vi "VIH HelpGen - Build Object Description for HTML.vi"(7 "Ena \"No Description\" message (F)":bool, 8 "Generate \"HTML Description\" (T)":bool=TRUE, 9 "Custom Description":string, 10 "Default Description":string, 11 "DscrMode":T2) -> (0 "HTML Tagset allowed":T1(ring), 2 "Description HTML out":string)   [LabVIEW 2014]
doc: "::: VI Helpeks :::\nCopyright (c) 2000-2026 Konstantin Shifershteyn. All rights reserved."
uses:
  _VIH HelpGen.llb/VIH HelpGen Typedef - Enum - Description Mode.ctl
panel:
  in  "Use Descripion Terminator (T)":bool=TRUE
  # "VI Helpeks\nCopyright (c) 2012-2026 Konstantin Shifershteyn"
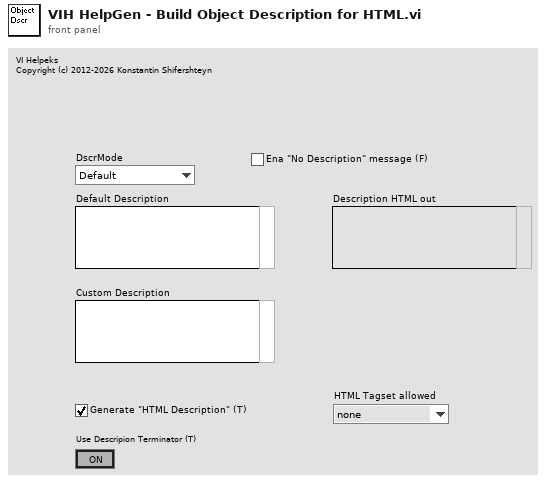
[diagram p1: front panel]
types:
  T1 = enum16{"none", "LV description", "VH minimum", "VH extended"}
  T2 = typedef "VIH HelpGen Typedef - Enum - Description Mode.ctl" = enum16{"Default", "Description", "Description1", "Description2", "Custom", "None"}
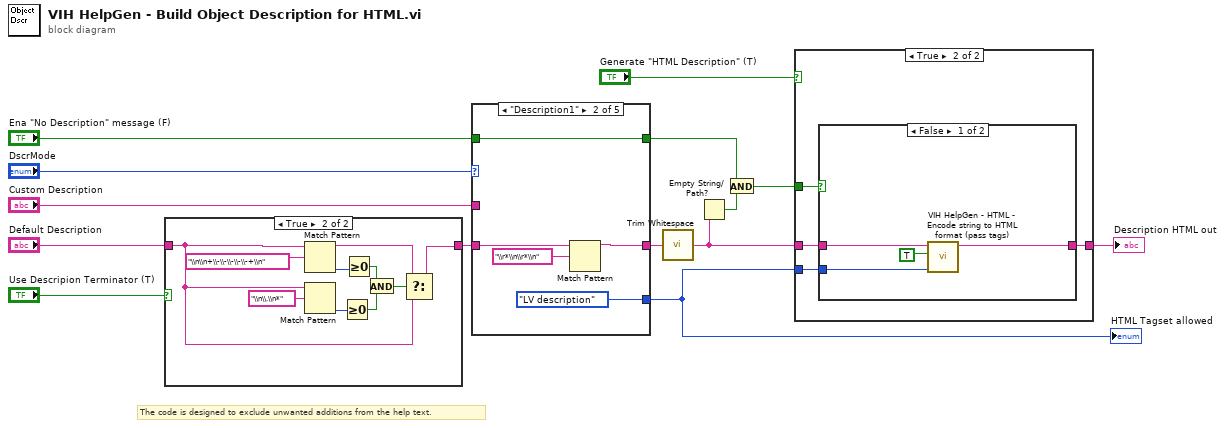
[diagram p0: block diagram]
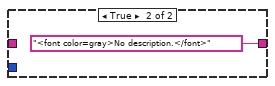
[diagram p4: hidden frame]
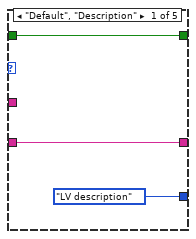
[diagram p5: hidden frame]
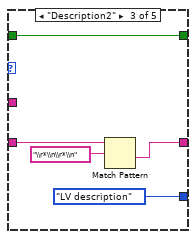
[diagram p6: hidden frame]
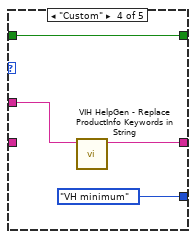
[diagram p7: hidden frame]
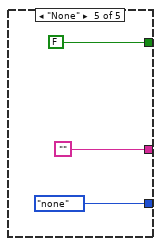
[diagram p8: hidden frame]
diagram:
  # "The code is designed to exclude unwanted additions from the help text."
  n1 = case shown="True" "Use Descripion Terminator (T)" {
    tunnel: "Default Description" -> [w15 w16]
    tunnel: [w15 w17] -> w2
    frame False {
    }
    frame True {
      n2 = Match Pattern(string=w16, regular expression="\\n\\n+\\-\\-\\-\\-\\-+\\n") -> (before substring=w19:string, offset past match=w23:i32)  [unwired: 1 in, 2 out]
      n3 = Match Pattern(string=w16, regular expression="\\n\\.\\n*") -> (offset past match=w22:i32)  [unwired: 1 in, 3 out]
      n4 = Greater Or Equal To 0?(x=w22) -> (x >= 0?=w20:bool)
      n5 = Greater Or Equal To 0?(x=w23) -> (x >= 0?=w21:bool)
      n6 = And(x=w21, y=w20) -> (x .and. y?=w18:bool)
      n7 = Select(t=w19, s=w18, f=w16) -> (s? t:f=w17:string)
    }
  }
  n8 = case shown="\"Description1\"" "DscrMode" {
    tunnel: w2 -> [w28 w33 w38 _ _]
    tunnel: [w28 w32 w35 w40 ""] -> w14
    tunnel: "Custom Description" -> [_ _ _ w39 _]
    tunnel: [w27 w31 w36 w42 FALSE] -> w7
    tunnel: "Ena \"No Description\" message (F)" -> [w27 w31 w36 w42 _]
    tunnel: [T1."LV description" ("Tag set") T1."LV description" ("Tag set") T1."LV description" ("Tag set") T1."VH minimum" ("Tag set") T1."none" ("Tag set")] -> w5
    frame "Default", "Description" {
    }
    frame "Description1" {
      n9 = Match Pattern(string=w33, regular expression="\\r*\\n\\r*\\n") -> (before substring=w32:string)  [unwired: 1 in, 3 out]
    }
    frame "Description2" {
      n10 = Match Pattern(string=w38, regular expression="\\r*\\n\\r*\\n") -> (after substring=w35:string)  [unwired: 1 in, 3 out]
    }
    frame "Custom" {
      n11 = call "VIH HelpGen - Replace ProductInfo Keywords in String.vi"("String in"=w39) -> ("String out"=w40:string)  [unwired: 10 in]
    }
    frame "None" {
    }
  }
  "HTML Tagset allowed" <- w5
  n12 = call <vilib>:"Trim Whitespace.vi"("string"=w14) -> ("trimmed string"=w8:string)  [unwired: 1 in]
  n13 = Empty String/Path?(string/path=w8) -> (empty?=w10:bool)
  n14 = And(x=w7, y=w10) -> (x .and. y?=w9:bool)
  n15 = case shown="True" "Generate \"HTML Description\" (T)" {
    tunnel: [w46 w50] -> w11
    tunnel: w9 -> [_ w49]
    tunnel: w8 -> [w46 w48]
    tunnel: w5 -> [_ w47]
    frame False {
    }
    frame True {
      n16 = case shown="False" w49 {
        tunnel: [w54 "<font color=gray>No description.</font>"] -> w50
        tunnel: w48 -> [w53 _]
        tunnel: w47 -> [w52 _]
        frame False {
          n17 = call "VIH HelpGen - HTML - Encode string to HTML format (pass tags).vi"("HTML Tagset allowed"=w52, "Reject CR (F)"=TRUE, "string"=w53) -> ("HTML string"=w54:string)  [unwired: 8 in]
        }
        frame True {
        }
      }
    }
  }
  "Description HTML out" <- w11
